vi "[ex ce] Scalar & Array processing speed.vi"() -> ()   [LabVIEW 2021]
doc: "<B>Run speed example</B>\n\nExample demonstrares advantage of polymorthism. CalcExpress VI can process the same data with the same formula much faster if it is called once with data passed in array instead of calling it multiple times for every data point.\n\n::: CalcExpress Toolkit :::\nCopyright (c) 2000-2026 Konstantin Shifershteyn. All rights reserved."
panel:
  in  "stop":bool
  out "graph2":cluster{dbl[], dbl[]}(graph)
  out "error2":bool caption="error"
  in  "exp2":string="x = sin(i+w) * sin(i/4);\ny = sin(i+w) * cos(i/4);"
  out "calctime 2":u32 caption="calc time, ms"
  out "graph1":cluster{dbl[], dbl[]}(graph)
  out "error1":bool caption="error"
  in  "exp1":string="x = sin(i+w) * sin(i/4);\ny = sin(i+w) * cos(i/4);\ni += 0.1;"
  out "calctime 1":u32 caption="calc time, ms"
  in  "N points":i32=10000
  # "processing  point by point"
  # "processing  array of points"
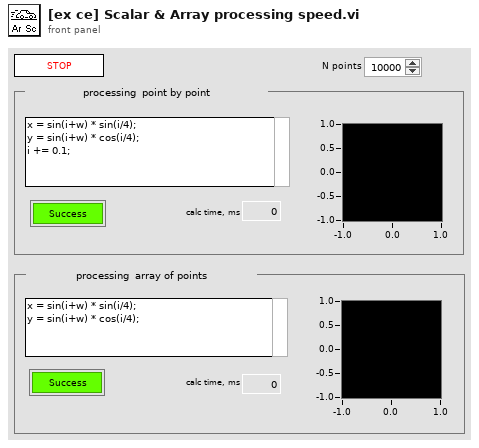
[diagram p1: front panel]
types:
  T1 = enum16{"create", "destroy", "set value", "get value"}
  T2 = typedef "VarMan Variable Context Handle.ctl" = i32
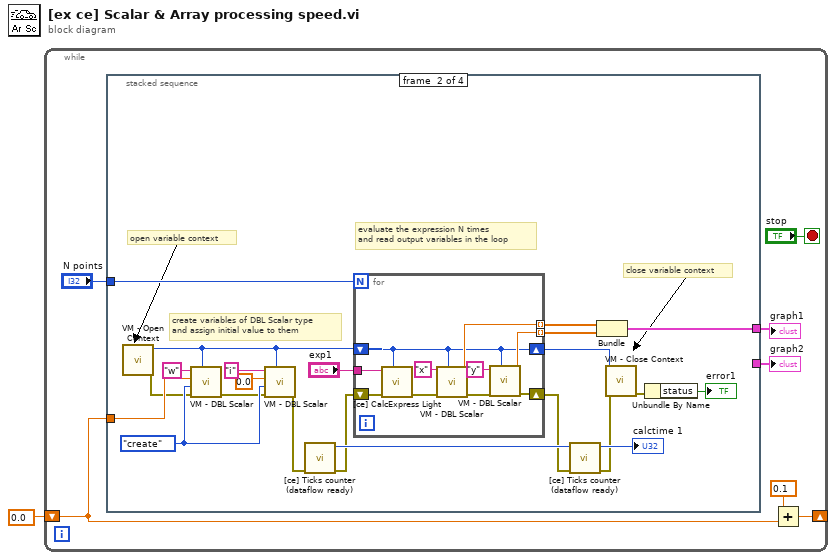
[diagram p0: block diagram]
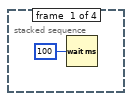
[diagram p2: hidden frame]
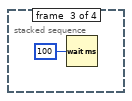
[diagram p3: hidden frame]
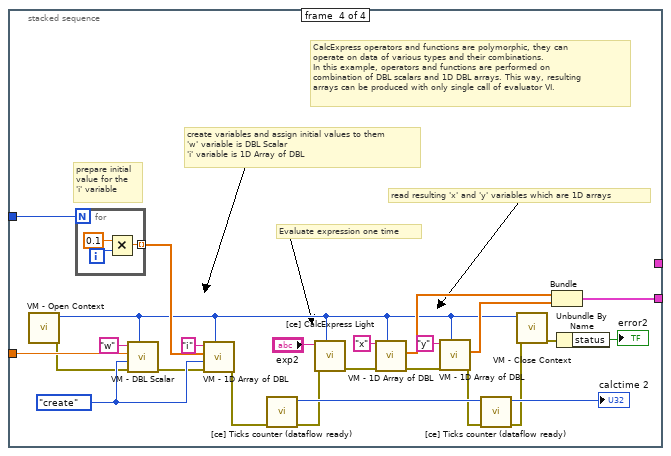
[diagram p4: hidden frame]
diagram:
  n1 = while {
    shift-left: 0.0 -> [w3]
    shift-right: [w5] -> _
    stop <- "stop" stop-if-true
    n2 = stacked-sequence "Sequence" {
      tunnel: "N points" -> [_ w25 _ w57]
      tunnel: [_ _ _ w60] -> w7
      tunnel: [_ w26 _ _] -> w6
      tunnel: w3 -> [_ w19 _ w55]
      frame #0 {
        n3 = Wait (ms)(milliseconds to wait=u32 100) -> ()  [unwired: 1 out]
      }
      frame #1 {
        w20 = T1."create" ("cmd")
        # "evaluate the expression N times\nand read output variables in the loop"
        # "close variable context"
        # "open variable context"
        # "create variables of DBL Scalar type\nand assign initial value to them"
        n4 = call "VM - Open Context.vi"() -> ("error out"=w18:errorcluster, "VC Handle out"=w10:T2)  [unwired: 9 in, 1 out]
        n5 = call "VM - DBL Scalar.vi"("VC Handle"=w10, "error in"=w18, "cmd"=w20, "value in"=w19, "name_spec"="w" ("name")) -> ("error out"=w17:errorcluster)  [unwired: 1 in, 5 out]
        n6 = call "VM - DBL Scalar.vi"("VC Handle"=w10, "error in"=w17, "cmd"=w20, "value in"=0.0 ("value (0)"), "name_spec"="i") -> ("error out"=w16:errorcluster)  [unwired: 1 in, 5 out]
        n7 = call "[ce] Ticks counter (dataflow ready).vi"("error in"=w16) -> ("error out"=w15:errorcluster, "ticks (current-input)"=w24:u32)  [unwired: 4 in, 3 out]
        n8 = for {
          N: w25 -> [_]
          tunnel: [w39] -> w29 mode=indexing
          tunnel: [w38] -> w30 mode=indexing
          shift-right: [w33] -> w14
          shift-left: w15 -> [w37]
          shift-right: [w32] -> w31
          shift-left: w10 -> [w32]
          tunnel: "exp1" -> [w36]
          n9 = call "[ce] CalcExpress Light.vi"("VC Handle"=w32, "error in"=w37, "expression"=w36) -> ("error out"=w35:errorcluster)  [unwired: 6 in, 2 out]
          n10 = call "VM - DBL Scalar.vi"("VC Handle"=w32, "error in"=w35, "name_spec"="x" ("var name")) -> ("error out"=w34:errorcluster, "value out"=w38:dbl)  [unwired: 3 in, 4 out]
          n11 = call "VM - DBL Scalar.vi"("VC Handle"=w32, "error in"=w34, "name_spec"="y" ("var name")) -> ("error out"=w33:errorcluster, "value out"=w39:dbl)  [unwired: 3 in, 4 out]
        }
        n12 = call "[ce] Ticks counter (dataflow ready).vi"("error in"=w14, "ticks in"=w24) -> ("error out"=w13:errorcluster, "ticks (current-input)"=→"calctime 1":u32)  [unwired: 3 in, 3 out]
        n13 = Bundle(w30, w29) -> (w26:cluster{dbl[], dbl[]})  [unwired: 1 in]
        n14 = call "VM - Close Context.vi"("error in"=w13, "VC Handle"=w31) -> ("error out"=w12:errorcluster)  [unwired: 8 in, 1 out]
        n15 = Unbundle By Name(w12) -> ("status"=→"error1":bool)
      }
      frame #2 {
        n16 = Wait (ms)(milliseconds to wait=u32 100) -> ()  [unwired: 1 out]
      }
      frame #3 {
        w54 = T1."create" ("cmd")
        # "create variables and assign initial values to them\n'w' variable is DBL Scalar\n'i' variable is 1D Array of DBL"
        # "Evaluate expression one time"
        # "read resulting 'x' and 'y' variables which are 1D arrays"
        # "prepare initial\nvalue for the\n'i' variable"
        # "CalcExpress operators and functions are polymorphic, they can\noperate on data of various types and their combinations.\nIn this example, operators and functions are performed on\ncombination of DBL scalars and 1D DBL arrays. This way, resulting\narrays can be produced with only single call of evaluator VI."
        n17 = call "VM - Open Context.vi"() -> ("error out"=w52:errorcluster, "VC Handle out"=w43:T2)  [unwired: 9 in, 1 out]
        n18 = for {
          N: w57 -> [_]
          tunnel: [w68] -> w65 mode=indexing
          i -> [w70]
          n19 = Multiply(x=0.1, y=w70) -> (x*y=w68:dbl)
        }
        n20 = call "VM - DBL Scalar.vi"("VC Handle"=w43, "error in"=w52, "cmd"=w54, "value in"=w55, "name_spec"="w" ("name")) -> ("error out"=w51:errorcluster)  [unwired: 1 in, 5 out]
        n21 = call "VM - 1D Array of DBL.vi"("VC Handle"=w43, "error in"=w51, "cmd"=w54, "value in"=w65, "name_spec"="i") -> ("error out"=w50:errorcluster)  [unwired: 1 in, 5 out]
        n22 = call "[ce] Ticks counter (dataflow ready).vi"("error in"=w50) -> ("error out"=w49:errorcluster, "ticks (current-input)"=w59:u32)  [unwired: 4 in, 3 out]
        n23 = call "[ce] CalcExpress Light.vi"("VC Handle"=w43, "error in"=w49, "expression"="exp2") -> ("error out"=w48:errorcluster)  [unwired: 6 in, 2 out]
        n24 = call "VM - 1D Array of DBL.vi"("VC Handle"=w43, "error in"=w48, "name_spec"="x" ("var name")) -> ("error out"=w47:errorcluster, "value out"=w44:dbl[])  [unwired: 3 in, 4 out]
        n25 = call "VM - 1D Array of DBL.vi"("VC Handle"=w43, "error in"=w47, "name_spec"="y" ("var name")) -> ("error out"=w46:errorcluster, "value out"=w67:dbl[])  [unwired: 3 in, 4 out]
        n26 = call "[ce] Ticks counter (dataflow ready).vi"("error in"=w46, "ticks in"=w59) -> ("error out"=w45:errorcluster, "ticks (current-input)"=→"calctime 2":u32)  [unwired: 3 in, 3 out]
        n27 = call "VM - Close Context.vi"("error in"=w45, "VC Handle"=w43) -> ("error out"=w61:errorcluster)  [unwired: 8 in, 1 out]
        n28 = Bundle("value out"=w44, "value out"=w67) -> (w60:cluster{"value out":dbl[], "value out":dbl[]})  [unwired: 1 in]
        n29 = Unbundle By Name(w61) -> ("status"=→"error2":bool)
      }
    }
    "graph2" <- w7
    "graph1" <- w6
    n30 = Add(x=0.1, y=w3) -> (x+y=w5:dbl)
  }
